vi "VIH HelpGen - Write HTML File - Common - Details.vi"(4 "Templates":T2, 6 "Details Params":cluster{"DetailsMode":T3, "DetailsText":string}, 7 "Save params":T1, 8 "error in":errorcluster, 9 "Original VI Name":string, 10 "HTML in":string, 11 "VI Reference":refnum<vi>) -> (0 "error out":errorcluster, 2 "HTML out":string, 3 "dup VI Reference":refnum<vi>)   [LabVIEW 2014]
doc: "::: VI Helpeks :::\nCopyright (c) 2000-2026 Konstantin Shifershteyn. All rights reserved."
uses:
  VIH HelpGen Typedef - Enum - Description Mode.ctl
  VIH HelpGen Typedef - Table Templates Cluster - VI Help.ctl
panel:
  # "VI Helpeks\nCopyright (c) 2012-2026 Konstantin Shifershteyn"
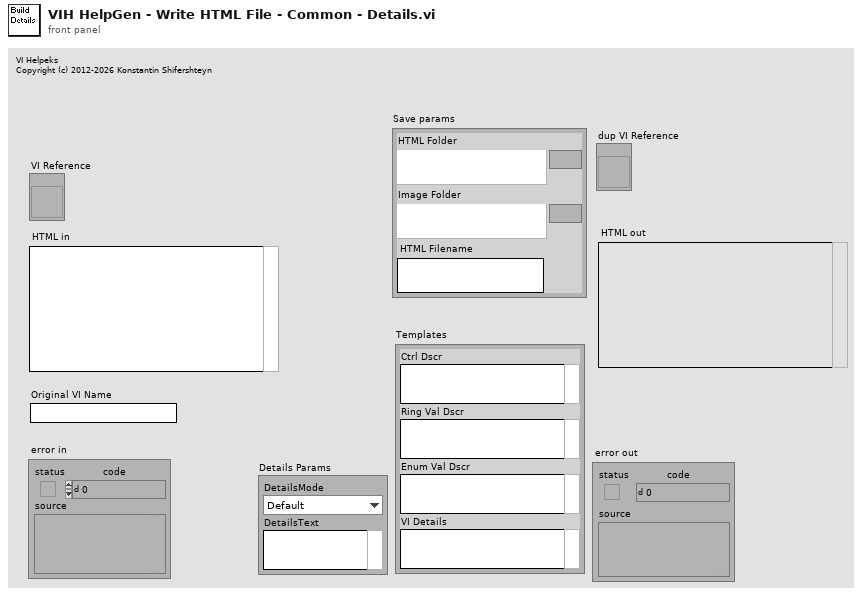
[diagram p1: front panel]
types:
  T1 = cluster{"HTML Folder":path, "Image Folder":path, "HTML Filename":string}
  T2 = typedef "VIH HelpGen Typedef - Table Templates Cluster - VI Help.ctl" = cluster{"Ctrl Dscr":string, "Ring Val Dscr":string, "Enum Val Dscr":string, "VI Details":string}
  T3 = typedef "VIH HelpGen Typedef - Enum - Description Mode.ctl" = enum16{"Default", "Description", "Description1", "Description2", "Custom", "None"}
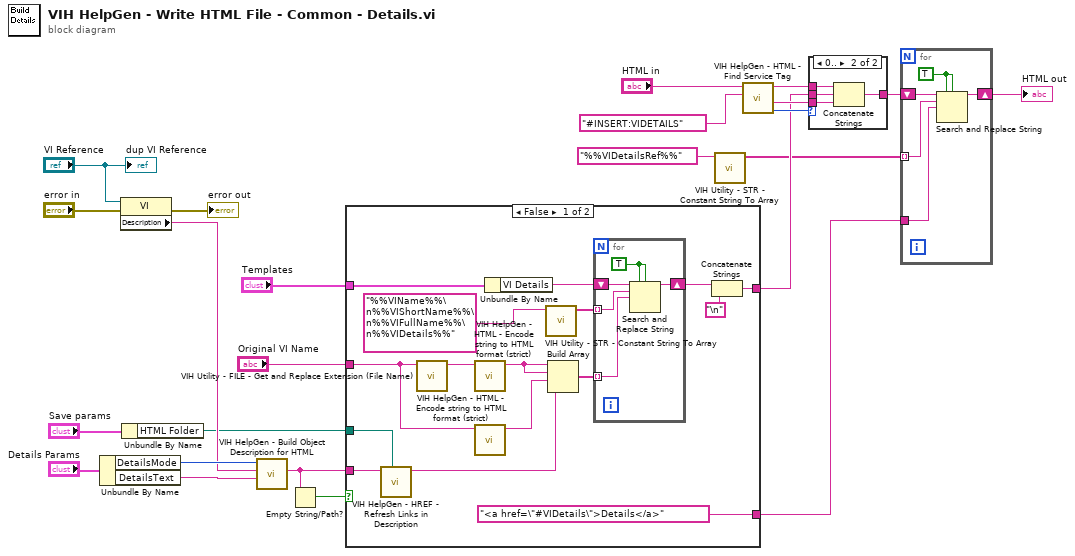
[diagram p0: block diagram]
diagram:
  n1 = Unbundle By Name("Details Params") -> ("DetailsMode"=w17:T3, "DetailsText"=w15:string)
  n2 = property class="VI"(reference="VI Reference", error in="error in") -> (error out=→"error out":errorcluster, "Description"=w16:string)  [unwired: 1 out]
  n3 = Unbundle By Name("Save params") -> ("HTML Folder"=w1:path)
  n4 = call "VIH HelpGen - Build Object Description for HTML.vi"("Custom Description"=w15, "Default Description"=w16, "DscrMode"=w17) -> ("Description HTML out"=w9:string)  [unwired: 7 in, 1 out]
  n5 = Empty String/Path?(string/path=w9) -> (empty?=w8:bool)
  n6 = case shown="False" w8 {
    tunnel: "Original VI Name" -> [w28 _]
    tunnel: "Templates" -> [w36 _]
    tunnel: [w30 _] -> w10
    tunnel: w9 -> [w33 _]
    tunnel: w1 -> [w32 _]
    tunnel: ["<a href=\"#VIDetails\">Details</a>" _] -> w3
    frame False {
      n7 = call "VIH HelpGen - HREF - Refresh Links in Description.vi"("HTML Folder"=w32, "Description in"=w33) -> ("Description out"=w37:string)  [unwired: 9 in]
      n8 = call "VIH Utility - FILE - Get and Replace Extension (File Name).vi"("File name"=w28) -> ("File name out"=w27:string)  [unwired: 9 in, 1 out]
      n9 = call "VIH HelpGen - HTML - Encode string to HTML format (strict).vi"("string"=w27) -> ("HTML string"=w25:string)  [unwired: 10 in]
      n10 = call "VIH HelpGen - HTML - Encode string to HTML format (strict).vi"("string"=w28) -> ("HTML string"=w26:string)  [unwired: 10 in]
      n11 = Unbundle By Name(w36) -> ("VI Details"=w35:string)
      n12 = call "VIH Utility - STR - Constant String To Array.vi"("String in"="%%VIName%%\n%%VIShortName%%\n%%VIFullName%%\n%%VIDetails%%") -> ("Array out"=w39:string[])  [unwired: 10 in]
      n13 = Build Array(w25, w25, w26, w37) -> (w38:string[])
      n14 = for {
        shift-right: [w44] -> w34
        shift-left: w35 -> [w45]
        tunnel: w39 -> [w42] mode=indexing
        tunnel: w38 -> [w41] mode=indexing
        w43 = TRUE
        n15 = Search and Replace String(replace all?=w43, case sensitive?=w43, input string=w45, search string=w42, replace string=w41) -> (result string=w44:string)  [unwired: 3 in, 3 out]
      }
      n16 = Concatenate Strings(w34, "\n") -> (w30:string)
    }
    frame True {
    }
  }
  n17 = call "VIH Utility - STR - Constant String To Array.vi"("String in"="%%VIDetailsRef%%") -> ("Array out"=w4:string[])  [unwired: 10 in]
  n18 = call "VIH HelpGen - HTML - Find Service Tag.vi"("Tag name"="#INSERT:VIDETAILS", "HTML in"="HTML in") -> ("Offset out"=w19:i32, "After"=w20:string, "Before"=w21:string)  [unwired: 6 in, 1 out]
  n19 = case shown="0.." w19 {
    tunnel: w21 -> [w46 w50]
    tunnel: w20 -> [_ w49]
    tunnel: [w46 w48] -> w7
    tunnel: w10 -> [_ w47]
    frame ..-1 {
    }
    frame 0.. {
      n20 = Concatenate Strings(w50, w47, w49) -> (w48:string)
    }
  }
  n21 = for {
    shift-right: [w54] -> w6
    shift-left: w7 -> [w55]
    tunnel: w4 -> [w52] mode=indexing
    tunnel: w3 -> [w51]
    w53 = TRUE
    n22 = Search and Replace String(replace all?=w53, case sensitive?=w53, input string=w55, search string=w52, replace string=w51) -> (result string=w54:string)  [unwired: 3 in, 3 out]
  }
  "HTML out" <- w6
  "dup VI Reference" <- "VI Reference"
